vi "WPI_ADI_IMU_AHRS_RoboBees.vi"(8 "Yaw Axis":enum16{"X", "Y", "Z"}(ring)=enum."Z", 9 "dt (s)":dbl, 10 "IMU Rates":T1) -> (0 "Yaw":dbl(knob) scale=-180.0..180.0, 1 "Roll":dbl(knob) scale=-180.0..180.0, 2 "Pitch":dbl(knob) scale=-90.0..90.0, 3 "Output":dbl[](array[numeric]))   [LabVIEW 2015, in "FRC ADI MXP IMU.lvlib"]
uses:
  FRC ADI MXP IMU.lvlib
panel:
  in  "Tilt Comp (Yaw)":bool
  in  "tau mag":dbl=0.04
  in  "tau acc":dbl=0.6
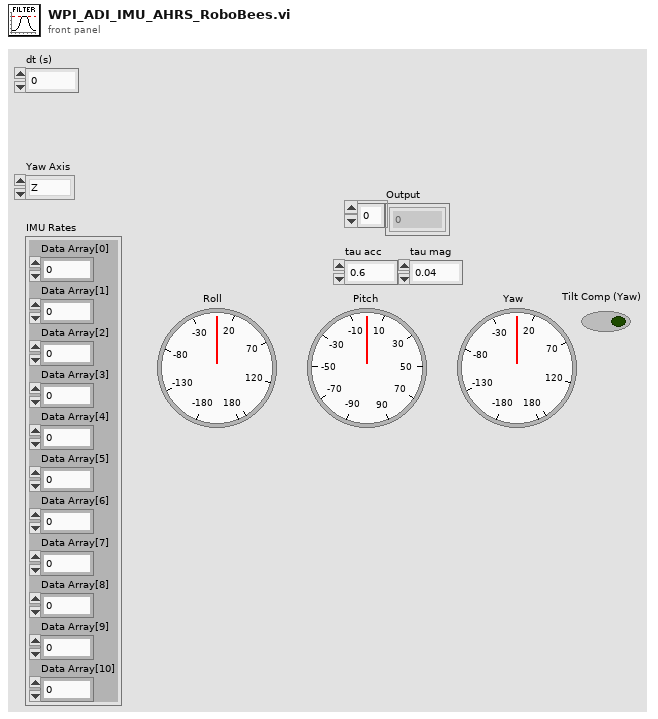
[diagram p1: front panel]
types:
  T1 = cluster{"Data Array[0]":dbl, "Data Array[1]":dbl, "Data Array[2]":dbl, "Data Array[3]":dbl, "Data Array[4]":dbl, "Data Array[5]":dbl, "Data Array[6]":dbl, "Data Array[7]":dbl, "Data Array[8]":dbl, "Data Array[9]":dbl, "Data Array[10]":dbl}
  T2 = cluster{"Xaccel":dbl, "Yaccel":dbl, "Zaccel":dbl}
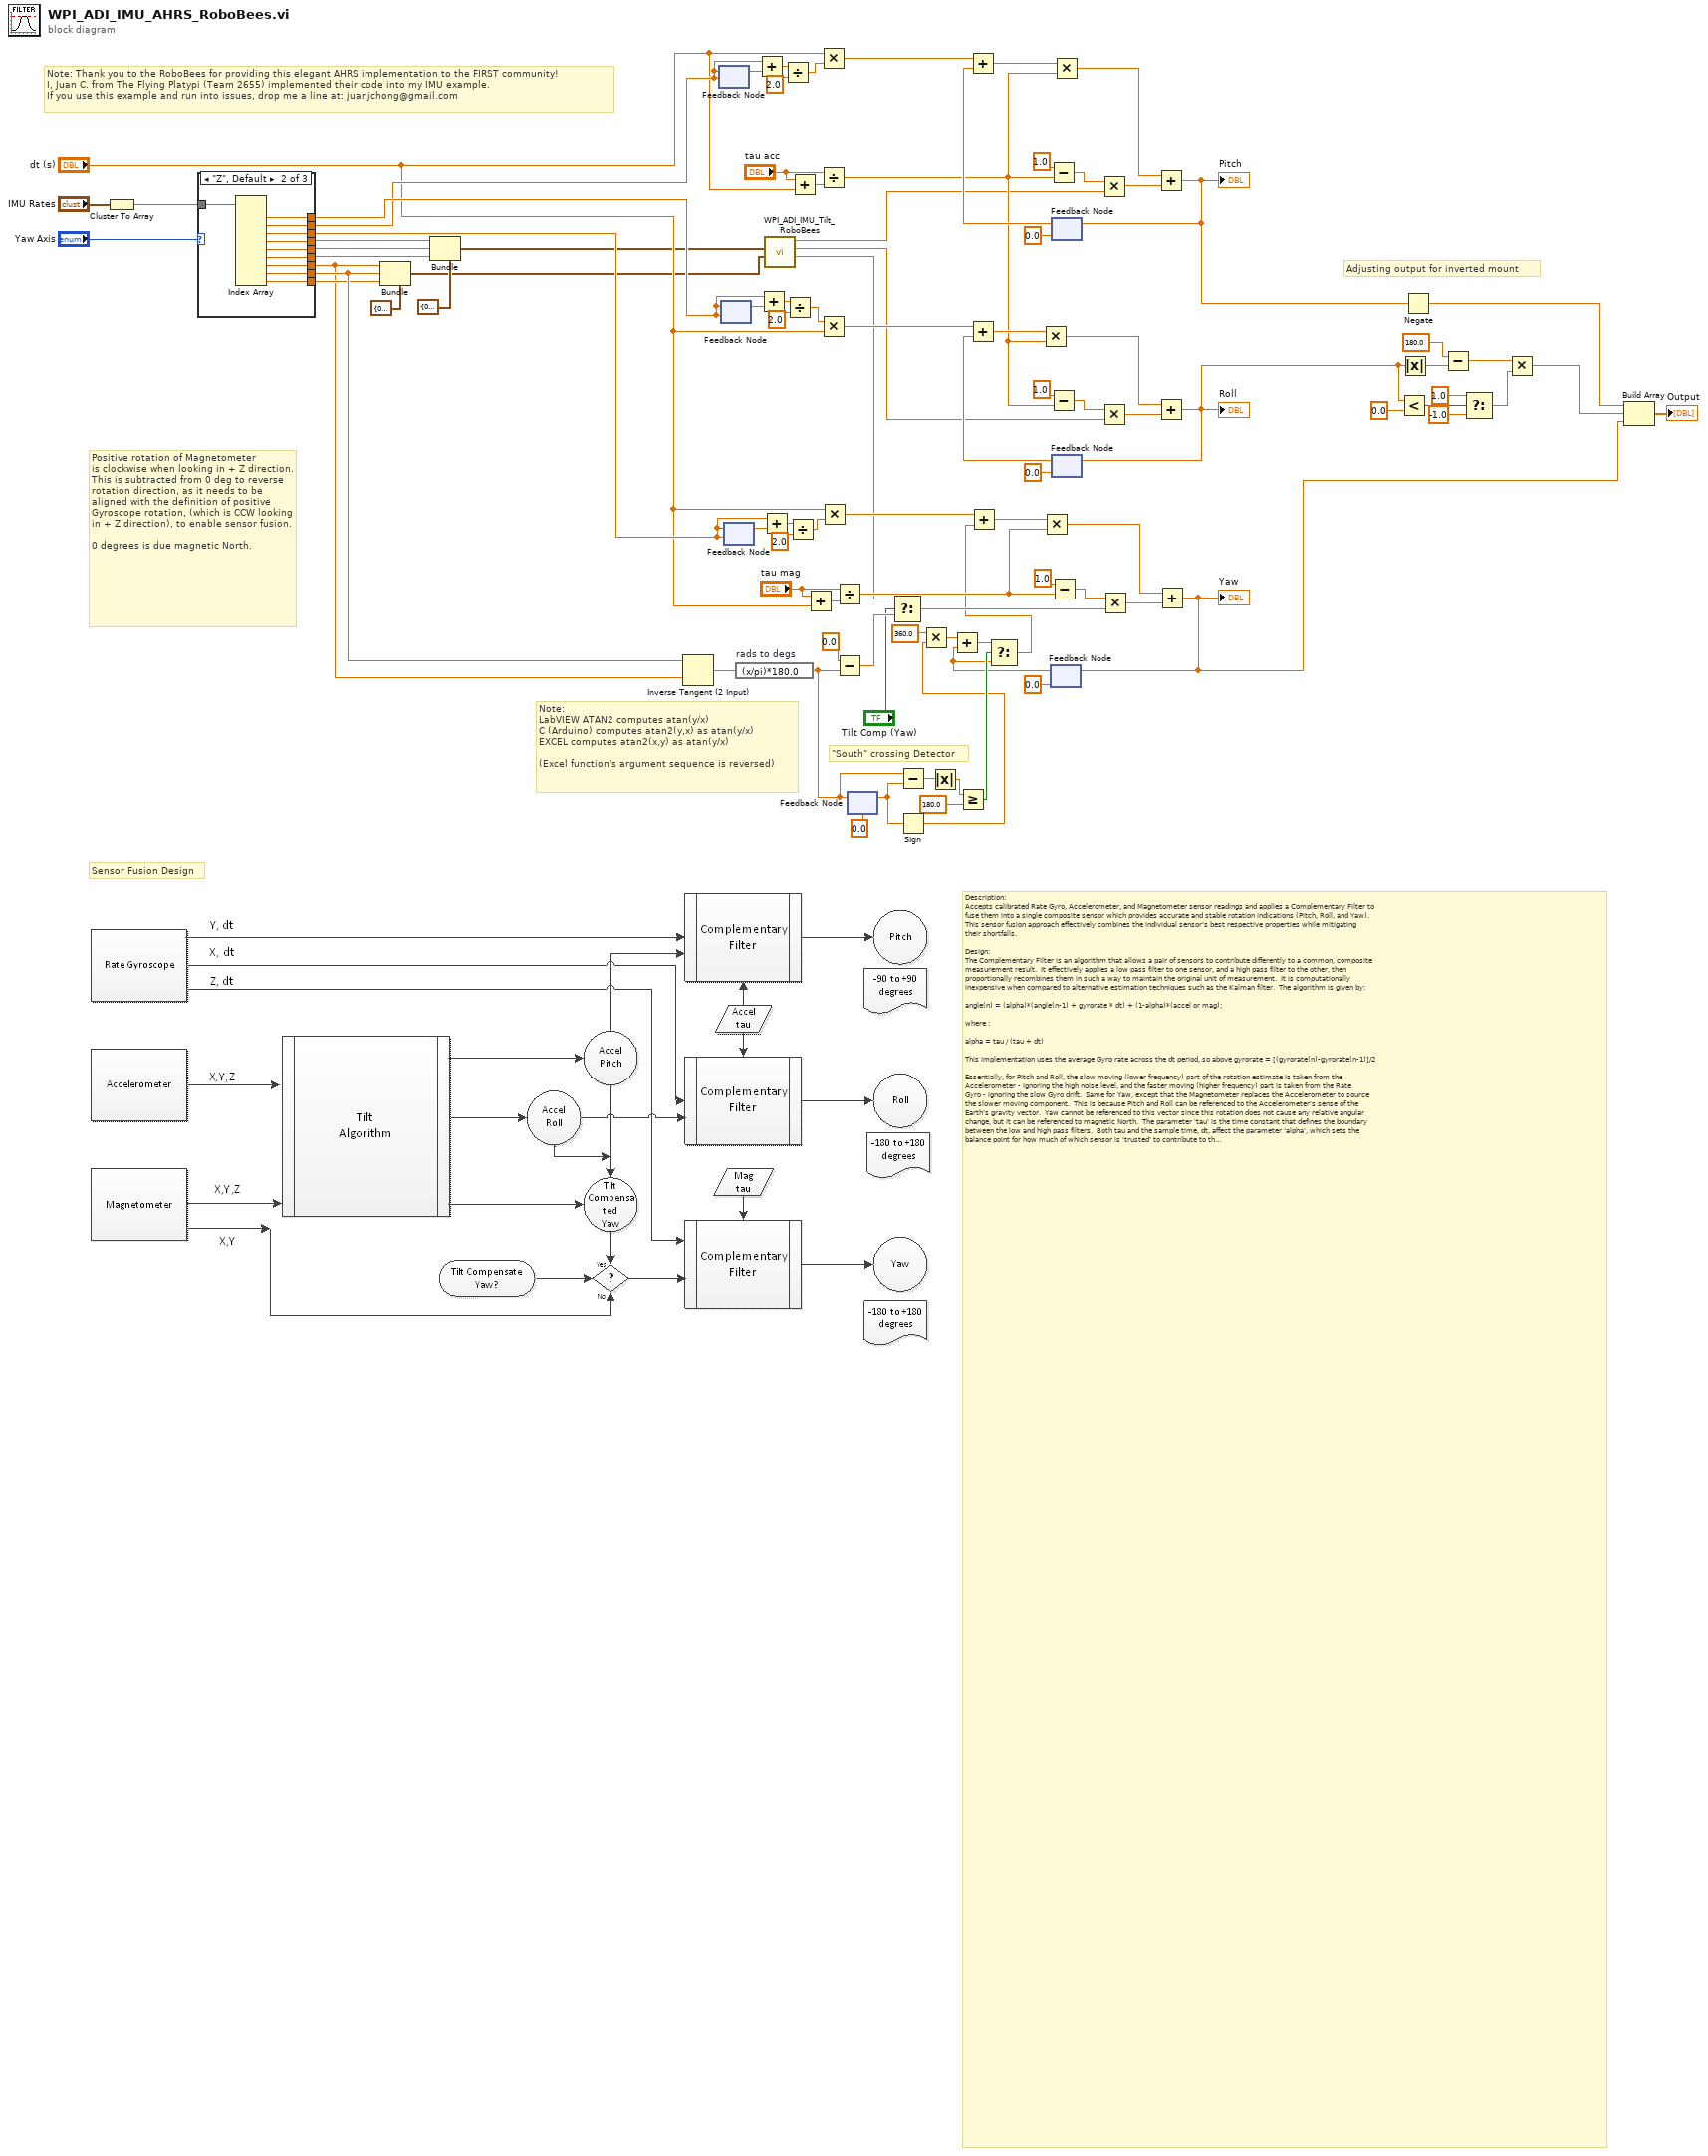
[diagram p0: block diagram]
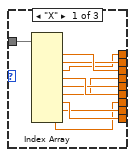
[diagram p2: hidden frame]
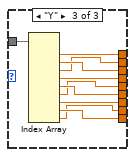
[diagram p3: hidden frame]
diagram:
  # "Note: Thank you to the RoboBees for providing this elegant AHRS implementation to the FIRST community!\nI, Juan C. from The Flying Platypi (Team 2655) implemented their code into my IMU example.\nIf you use this example and run into issues, drop me a line at: juanjchong@gmail.com"
  # "Adjusting output for inverted mount"
  # "Sensor Fusion Design"
  # "Description:\nAccepts calibrated Rate Gyro, Accelerometer, and Magnetometer sensor readings and applies a Complementary Filter to\nfuse them into a single composite sensor which provides accurate and stable rotation indications (Pitch, Roll, and Yaw).\nThis sensor fusion approach effectively combines the individual sensor's best respective properties while mitigating\ntheir shortfalls.\n\nDesign:\nThe Complementary Filter is an algorithm that allows a pair of sensors to contribute differently to a common, composite\nmeasurement result.  It effectively applies a low pass filter to one sensor, and a high pass filter to the other, then\nproportionally recombines them in such a way to maintain the original unit of measurement.  It is computationally\ninexpensive when compared to alternative estimation techniques such as the Kalman filter.  The algorithm is given by:\n\nangle(n) = (alpha)*(angle(n-1) + gyrorate * dt) + (1-alpha)*(accel or mag);\n\nwhere : \n\nalpha = tau / (tau + dt)\n\nThis implementation uses the average Gyro rate across the dt period, so above gyrorate = [(gyrorate(n)-gyrorate(n-1)]/2\n\nEssentially, for Pitch and Roll, the slow moving (lower frequency) part of the rotation estimate is taken from the\nAccelerometer - ignoring the high noise level, and the faster moving (higher frequency) part is taken from the Rate \nGyro - ignoring the slow Gyro drift.  Same for Yaw, except that the Magnetometer replaces the Accelerometer to source\nthe slower moving component.  This is because Pitch and Roll can be referenced to the Accelerometer's sense of the\nEarth's gravity vector.  Yaw cannot be referenced to this vector since this rotation does not cause any relative angular\nchange, but it can be referenced to magnetic North.  The parameter 'tau' is the time constant that defines the boundary\nbetween the low and high pass filters.  Both tau and the sample time, dt, affect the parameter 'alpha', which sets the\nbalance point for how much of which sensor is 'trusted' to contribute to the rotation estimate.\n\nThe Complementary Filter algorithm is applied to each X/Y/Z rotation axis to compute R/P/Y outputs, respectively.\n\nMagnetometer readings are tilt-compensated when Tilt-Comp-(Yaw) is asserted (True), by the IMU TILT subVI.  This\ncreates what is known as a tilt-compensated compass, which allows Yaw to be insensitive to the effects of a\nnon-level sensor, but generates error in Yaw during movement (coordinate acceleration).\n\nThe Yaw \"South\" crossing detector is necessary to allow a smooth transition across the +/- 180 deg discontinuity (inherent\nin the ATAN function).  Since -180 deg is congruent with +180 deg, Yaw needs to jump between these values when\ncrossing South (North is 0 deg).  The design depends upon comparison of successive Yaw readings to detect a cross-over\nevent.  The cross-over detector monitors the current reading and evaluates how far it is from the previous reading.  If it\nis greater than the previous reading by the Discriminant (= 180 deg), then Yaw just crossed South.\n\nBy choosing 180 as the Discriminant, the only way the detector can produce a false positive, assuming a loop iteration\nof 70 msec, is for it to rotate >2,571 dps ... (2,571=180/.07).  This is faster than the ST L3GD20 Gyro can register.  The\ndetector produces a Boolean True upon detecting a South crossing.  This is used to alter the (n-1) Yaw which was\npreviously stored, either adding or subtracting 360 degrees as required to place the previous Yaw in the correct quadrant\nwhenever crossing occurs.  The Modulus function cannot be used here as the Complementary Filter algorithm has 'state'\n(needs to remember previous Yaw).\n \nWe are in effect stitching together two ends of a ruler for 'modular arithmetic' (clock math).\n\nInputs:\nGYRO - Gyro rate and sample time measurements.\nACCEL - Acceleration measurements.\nMAG - Magnetic measurements.\nTAU ACC - tau parameter used to set sensor balance between Accel and Gyro for Roll and Pitch.\nTAU MAG -  tau parameter used to set sensor balance between Mag and Gyro for Yaw.\nTILT COMP (Yaw) - Enables Yaw tilt-compensation if True.\n\nOutputs:\nROLL - Filtered Roll about sensor X-axis.\nPITCH - Filtered Pitch about sensor Y-axis.\nYAW - Filtered Yaw about sensor Z-axis.\n\nVI Properties:\nExecution Reentrancy is set to Non Reentrant Execution\n\nImplementation:\nIt's best to establish the optimum loop sample time first.  See IMU READ implementation notes for guidance.  Each\ntau parameter should then be adjusted to achieve optimum sensor fusion.  tau acc affects Roll and Pitch, tau mag affects\nYaw.  Start at value 1 or 2 and decrease by half each time until the result doesn't drift, but not so far that the result gets\nnoisy.  An optimum tau for this IMU is likely in the range of 1.0 to 0.01, for a loop sample time between 10 and 100 ms.\n\nNote that both sample timing (dt) and tau both affect the balance parameter, 'alpha'.  Adjusting either dt or tau will\nrequire the other to be readjusted to maintain a particular filter performance.\n\nIt is likely best to set Yaw tilt-compensation to off (False) if the Yaw value is to be used as feedback in a closed loop\ncontrol application.  The tradeoff is that Yaw will only be accurate while the robot is level.\n\nSince a Yaw of -180 degrees is congruent with +180 degrees (they represent the same direction), it is possible that the\nYaw output will oscillate between these two values when the sensor happens to be pointing due South, as sensor\nnoise causes slight variation.  You will need to account for this possibility if you are using the Yaw value for decision-\nmaking in code.\n\n----- The RoboBees FRC Team 836! -----  Complement your passion to solve problems with a STEM Education!"
  # "\"South\" crossing Detector"
  # "Positive rotation of Magnetometer\nis clockwise when looking in + Z direction.  This is subtracted from 0 deg to reverse rotation direction, as it needs to be aligned with the definition of positive Gyroscope rotation, (which is CCW looking in + Z direction), to enable sensor fusion.\n\n0 degrees is due magnetic North."
  # "Note:\nLabVIEW ATAN2 computes atan(y/x)\nC (Arduino) computes atan2(y,x) as atan(y/x)\nEXCEL computes atan2(x,y) as atan(y/x)\n\n(Excel function's argument sequence is reversed)"
  n1 = Cluster To Array(cluster="IMU Rates") -> (array=w32:dbl[])
  n2 = case shown="\"Z\", Default" "Yaw Axis" {
    tunnel: [w100 w113 w122] -> w31
    tunnel: [w97 w112 w119] -> w23
    tunnel: w32 -> [w103 w111 w123]
    tunnel: [w94 w110 w116] -> w25
    tunnel: [w98 w109 w117] -> w22
    tunnel: [w99 w108 w118] -> w21
    tunnel: [w101 w107 w120] -> w30
    tunnel: [w102 w106 w121] -> w29
    tunnel: [w95 w105 w114] -> w27
    tunnel: [w96 w104 w115] -> w26
    frame "X" {
      n3 = Index Array(array=w103) -> (element #1=w102:dbl, element #2=w101:dbl, element #3=w100:dbl, element #4=w99:dbl, element #5=w98:dbl, element #6=w97:dbl, element #7=w96:dbl, element #8=w95:dbl, element #9=w94:dbl)  [unwired: 9 in]
    }
    frame "Z", Default {
      n4 = Index Array(array=w111) -> (element #1=w113:dbl, element #2=w107:dbl, element #3=w106:dbl, element #4=w112:dbl, element #5=w109:dbl, element #6=w108:dbl, element #7=w110:dbl, element #8=w105:dbl, element #9=w104:dbl)  [unwired: 9 in]
    }
    frame "Y" {
      n5 = Index Array(array=w123) -> (element #1=w122:dbl, element #2=w121:dbl, element #3=w120:dbl, element #4=w119:dbl, element #5=w118:dbl, element #6=w117:dbl, element #7=w116:dbl, element #8=w115:dbl, element #9=w114:dbl)  [unwired: 9 in]
    }
  }
  n6 = Bundle(cluster=cluster{"Xmag":dbl, "Ymag":dbl, "Zmag":dbl} {"Xmag"=0.0, "Ymag"=0.0, "Zmag"=0.0} ("Mag"), "Xmag"=w25, "Ymag"=w27, "Zmag"=w26) -> (w18:cluster{"Xmag":dbl, "Ymag":dbl, "Zmag":dbl})
  n7 = Bundle(cluster=T2 {"Xaccel"=0.0, "Yaccel"=0.0, "Zaccel"=0.0} ("Accel"), "Xaccel"=w23, "Yaccel"=w22, "Zaccel"=w21) -> (w19:T2)
  n8 = Inverse Tangent (2 Input)(1:w25, 2:w27) -> (0:w66:dbl)
  n9 = feedback #1(w30) -> (w55:dbl)
  n10 = feedback-in #1(w30) -> ()
  n11 = feedback #2(w31) -> (w49:dbl)
  n12 = feedback-in #2(w31) -> ()
  n13 = feedback #3(w29) -> (w47:dbl)
  n14 = feedback-in #3(w29) -> ()
  n15 = expression code="(x/pi)*180.0" "rads to degs"(w66) -> (w36:dbl)
  n16 = Add(x=w30, y=w55) -> (x+y=w54:dbl)
  n17 = Add(x=w31, y=w49) -> (x+y=w50:dbl)
  n18 = Add(x=w29, y=w47) -> (x+y=w46:dbl)
  n19 = call "WPI_ADI_IMU_Tilt_RoboBees.vi"("Mag"=w18, "Accel"=w19) -> ("Yaw"=w15:dbl, "Roll"=w16:dbl, "Pitch"=w17:dbl)  [unwired: 6 in, 1 out]
  n20 = Divide(x=w54, y=2.0) -> (x/y=w52:dbl)
  n21 = Divide(x=w50, y=2.0) -> (x/y=w48:dbl)
  n22 = Divide(x=w46, y=2.0) -> (x/y=w44:dbl)
  n23 = Add(x="tau acc", y="dt (s)") -> (x+y=w92:dbl)
  n24 = Add(x="tau mag", y="dt (s)") -> (x+y=w67:dbl)
  n25 = Multiply(x="dt (s)", y=w52) -> (x*y=w80:dbl)
  n26 = Divide(x="tau acc", y=w92) -> (x/y=w76:dbl)
  n27 = Multiply(x=w48, y="dt (s)") -> (x*y=w90:dbl)
  n28 = Multiply(x="dt (s)", y=w44) -> (x*y=w60:dbl)
  n29 = Divide(x="tau mag", y=w67) -> (x/y=w59:dbl)
  n30 = Subtract(x=0.0 ("y"), y=w36) -> (x-y=w63:dbl)
  n31 = feedback #4(0.0) -> (w37:dbl)
  n32 = feedback-in #4(w36) -> ()
  n33 = Select(t=w15, s="Tilt Comp (Yaw)", f=w63) -> (s? t:f=w64:dbl)
  n34 = Subtract(x=w36, y=w37) -> (x-y=w43:dbl)
  n35 = Sign(1:w37) -> (0:w39:dbl)
  n36 = Multiply(x=360.0 ("y"), y=w39) -> (x*y=w35:dbl)
  n37 = Absolute Value(x=w43) -> (abs(x)=w42:dbl)
  n38 = Greater Or Equal?(x=w42, y=180.0) -> (x >= y?=w40:bool)
  n39 = Subtract(x=1.0, y=w76) -> (x-y=w79:dbl)
  n40 = Subtract(x=1.0, y=w76) -> (x-y=w75:dbl)
  n41 = Subtract(x=1.0, y=w59) -> (x-y=w73:dbl)
  n42 = feedback #5(0.0) -> (w34:dbl)
  n43 = Add(x=w35, y=w34) -> (x+y=w56:dbl)
  n44 = Select(t=w56, s=w40, f=w34) -> (s? t:f=w57:dbl)
  n45 = Add(x=w60, y=w57) -> (x+y=w70:dbl)
  n46 = Multiply(x=w70, y=w59) -> (x*y=w72:dbl)
  n47 = feedback #6(0.0) -> (w84:dbl)
  n48 = Add(x=w80, y=w84) -> (x+y=w81:dbl)
  n49 = Multiply(x=w81, y=w76) -> (x*y=w83:dbl)
  n50 = feedback #7(0.0) -> (w74:dbl)
  n51 = Add(x=w90, y=w74) -> (x+y=w89:dbl)
  n52 = Multiply(x=w89, y=w76) -> (x*y=w87:dbl)
  n53 = Multiply(x=w79, y=w17) -> (x*y=w82:dbl)
  n54 = Multiply(x=w75, y=w16) -> (x*y=w88:dbl)
  n55 = Multiply(x=w73, y=w64) -> (x*y=w71:dbl)
  n56 = Add(x=w83, y=w82) -> (x+y=w4:dbl)
  "Pitch" <- w4
  n57 = feedback-in #6(w4) -> ()
  n58 = Add(x=w87, y=w88) -> (x+y=w3:dbl)
  "Roll" <- w3
  n59 = feedback-in #7(w3) -> ()
  n60 = Add(x=w72, y=w71) -> (x+y=w5:dbl)
  "Yaw" <- w5
  n61 = feedback-in #5(w5) -> ()
  n62 = Less?(x=w3, y=0.0) -> (x < y?=w10:bool)
  n63 = Absolute Value(x=w3) -> (abs(x)=w13:dbl)
  n64 = Negate(x=w4) -> (-x=w2:dbl)
  n65 = Subtract(x=180.0 ("y"), y=w13) -> (x-y=w7:dbl)
  n66 = Select(t=1.0, s=w10, f=-1.0) -> (s? t:f=w6:dbl)
  n67 = Multiply(x=w7, y=w6) -> (x*y=w1:dbl)
  n68 = Build Array(w2, w1, w5) -> (→"Output":dbl[])
